vi "Set_Get_FVG - Mode.vi"(8 "error out":errorcluster, 10 "?":T1, 11 "Enum":T2) -> (0 "error out 2":errorcluster, 3 "Enum":T1)   [LabVIEW 2021]
uses:
  Control/Set_Get.ctl
  Control/Mode.ctl
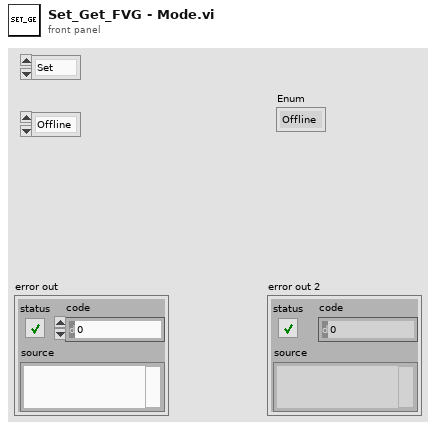
[diagram p1: front panel]
types:
  T1 = typedef "Mode.ctl" = enum16{"Offline", "Online"}
  T2 = typedef "Set_Get.ctl" = enum16{"Set", "Get"}
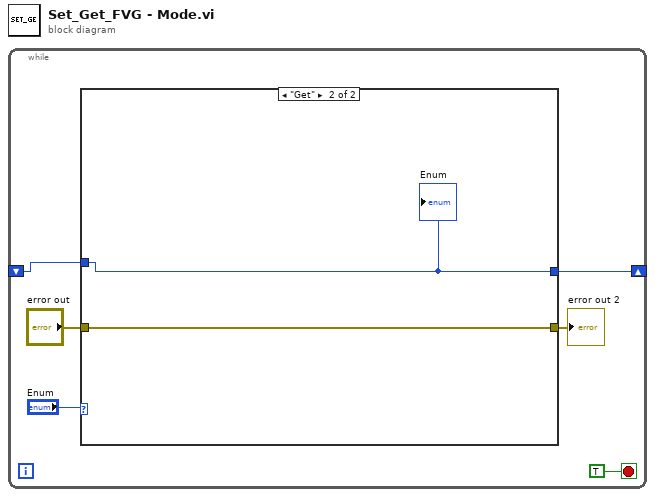
[diagram p0: block diagram]
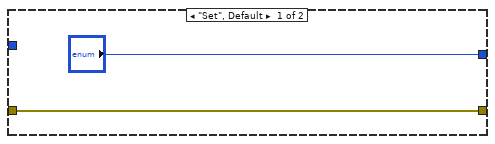
[diagram p2: hidden frame]
diagram:
  n1 = while {
    shift-right: [w2] -> _
    shift-left: _ -> [w1]
    stop <- TRUE stop-if-true
    n2 = case shown="\"Get\"" "Enum" {
      tunnel: [w8 w10] -> w3
      tunnel: "error out" -> [w8 w10]
      tunnel: ["?" w9] -> w2
      tunnel: w1 -> [_ w9]
      frame "Set", Default {
      }
      frame "Get" {
        "Enum" <- w9
      }
    }
    "error out 2" <- w3
  }
